vi "set NR UL_DL Center Channel Number.vi"(8 "error in (no error)":errorcluster, 9 "Direction":T1, 10 "Center Channel Argements":T2, 11 "Anritsu Call Box_Implement in":refnum<class "Anritsu Call Box_Implement.lvclass">) -> (0 "error out":errorcluster, 3 "Anritsu Call Box_Implement out":refnum<class "Anritsu Call Box_Implement.lvclass">)   [LabVIEW 2023, in "ANRITSU Call Box.lvlib" / "Anritsu Call Box_Implement.lvclass"]
uses:
  Anritsu Call Box_Implement.lvclass
  Anritsu Call Box_Implement.lvclass/Anritsu Call Box_Implement.ctl
  NR/NR.lvclass
  Type Definition/NR Center Channel Arguments.ctl
  ANRITSU Call Box.lvlib
  Type Definition/Uplink Downlink Enum.ctl
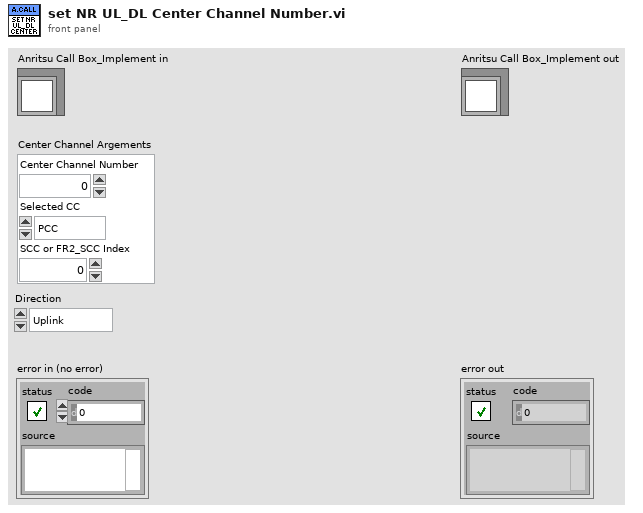
[diagram p1: front panel]
types:
  T1 = typedef "ANRITSU Call Box.lvlib/Uplink Downlink Enum.ctl" = enum16{"Uplink", "Downlink"}
  T2 = typedef "ANRITSU Call Box.lvlib/NR Center Channel Arguments.ctl" = cluster{"Center Channel Number":u32, "Selected CC":enum16{"PCC", "SCC", "FR2_PCC", "FR2_SCC"}, "SCC or FR2_SCC Index":u32}
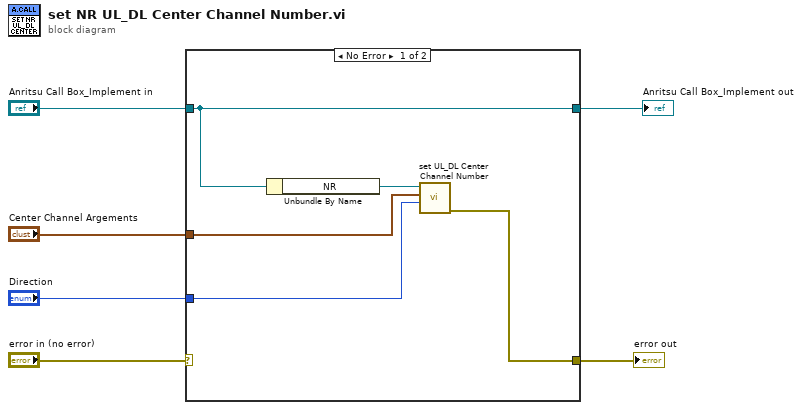
[diagram p0: block diagram]
diagram:
  n1 = case shown="No Error" "error in (no error)" {
    selector: "error in (no error)" -> [_ w12]
    tunnel: "Anritsu Call Box_Implement in" -> [w11 w13]
    tunnel: [w11 w13] -> w5
    tunnel: [w7 w12] -> w3
    tunnel: "Direction" -> [w9 _]
    tunnel: "Center Channel Argements" -> [w8 _]
    frame No Error {
      n2 = Unbundle By Name(w11) -> ("NR"=w10:refnum<class "NR.lvclass">)
      n3 = call "set UL_DL Center Channel Number.vi"("Direction"=w9, "Center Channel Argements"=w8, "NR in"=w10) -> ("error out"=w7:errorcluster)  [unwired: 7 in, 1 out]
    }
    frame Error {
    }
  }
  "error out" <- w3
  "Anritsu Call Box_Implement out" <- w5
